vi "test_input_required_result_multi_round.vi"(8 "error in":errorcluster) -> (0 "error out":errorcluster, 3 "text":string)   [LabVIEW 2020, in "Conformance MCP Server.lvlib"]
doc: "Conformance fixture (scenario input-required-result-multi-round). Takes no arguments and asks the user two questions in two rounds with Ask User.vi: first the key step1 (\"Step 1: What is your name?\", a form with the string name), and once that is answered the key step2 (\"Step 2: What is your favorite color?\", a form with the string color). With both answers text is \"Hello, <name>! Your favorite color is <color>.\". While an answer is missing it returns at once and text says which step is open."
uses:
  Conformance MCP Server.lvlib
  <vilib>/JDP Science/JSONtext/Next JSON Value.vi
  <vilib>/JDP Science/JSONtext/String Subset.vi
  <vilib>/JDP Science/JSONtext/support/Strip Quotes and Unescape.vi
  <vilib>/JDP Science/JSONtext/Parsing/Advance past next JSON Value (inlined COPY).vi
  <vilib>/JDP Science/JSONtext/support/Unescape JSON string.vi
  <vilib>/JDP Science/JSONtext/Parsing/Advance past whitespace.vi
  <vilib>/JDP Science/JSONtext/Parsing/Advance past String.vi
  <vilib>/JDP Science/JSONtext/Parsing/Advance past Number.vi
  <vilib>/JDP Science/JSONtext/Parsing/Advance past Line Ending.vi
  <vilib>/JDP Science/JSONtext/Parsing/Parse Full Path or Item Name.vi
  <vilib>/JDP Science/JSONtext/Parsing/Advance past Array.vi
  <vilib>/JDP Science/JSONtext/Parsing/Advance past Object.vi
  <vilib>/JDP Science/JSONtext/support/Error Cluster From Code.vi
  <vilib>/JDP Science/JSONtext/Offset/Find Item Locations by Path.vi
  <vilib>/JDP Science/JSONtext/Parsing/Advance past next JSON Value.vi
  src/MCP Server/MCP Server.lvlib
  <vilib>/JDP Science/JSONtext/JSONtext.lvlib
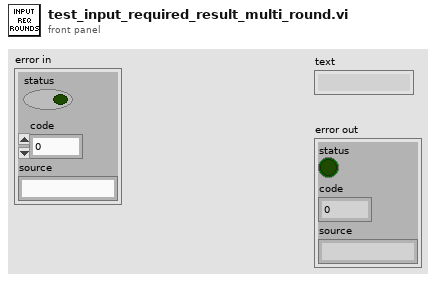
[diagram p1: front panel]
types:
  T1 = enum16{"accept", "decline", "cancel", "pending", "not supported"}
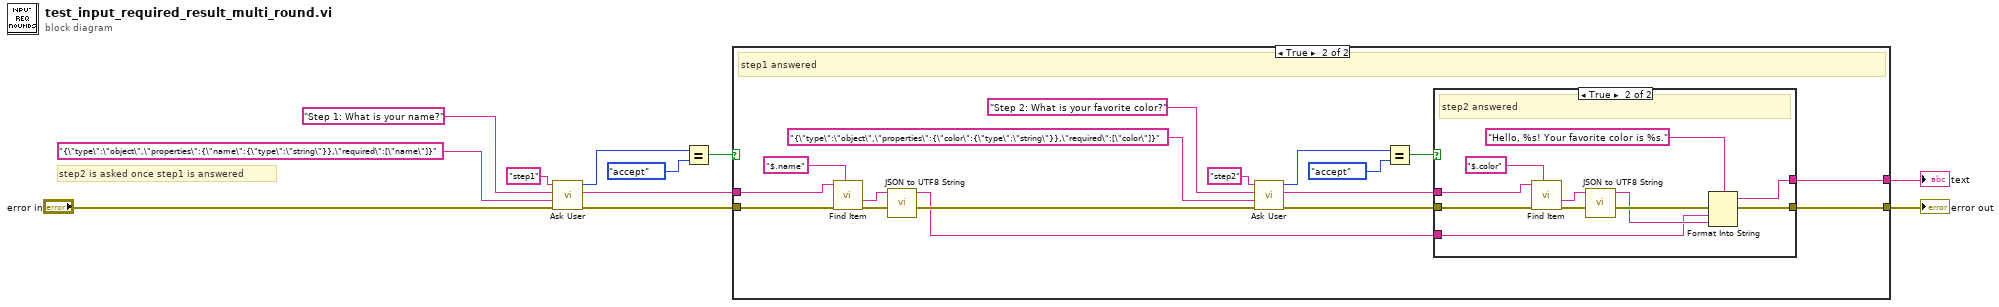
[diagram p0: block diagram]
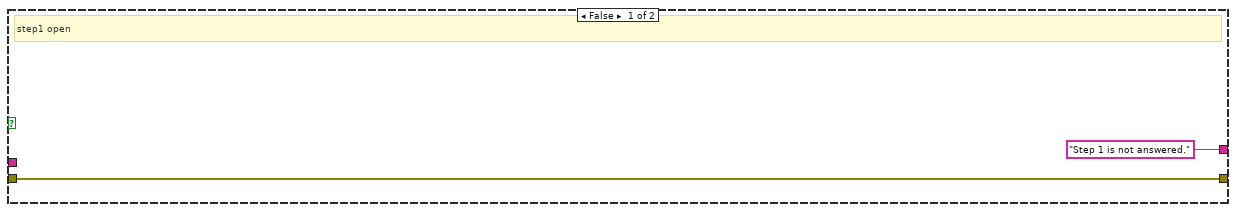
[diagram p2: hidden frame]
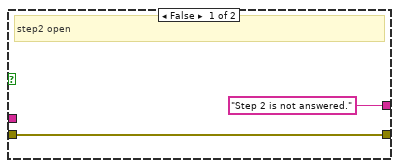
[diagram p3: hidden frame]
diagram:
  # "step2 is asked once step1 is answered"
  n1 = call "Ask User.vi"("error in"="error in", "requestedSchema"="{\"type\":\"object\",\"properties\":{\"name\":{\"type\":\"string\"}},\"required\":[\"name\"]}", "message"="Step 1: What is your name?", "key"="step1") -> ("error out"=w7:errorcluster, "content"=w6:string, "action"=w5:T1)  [unwired: 5 in]
  n2 = Equal?(x=w5, y=T1."accept" ("accept")) -> (x = y?=w9:bool)
  n3 = case shown="True" w9 {
    tunnel: w6 -> [_ w14]
    tunnel: w7 -> [w12 w15]
    tunnel: ["Step 1 is not answered." ("text") w29] -> w10
    tunnel: [w12 w30] -> w11
    frame False {
      # "step1 open"
    }
    frame True {
      # "step1 answered"
      n4 = call <vilib>:"Find Item.vi"("$Path or Item Name"="$.name", "error in (no error)"=w15, "JSON"=w14) -> ("error out"=w17:errorcluster, "<JSON>"=w18:string)  [unwired: 5 in, 2 out]
      n5 = call <vilib>:"JSON to UTF8 String.vi"("error in (no error)"=w17, "JSON"=w18) -> ("error out"=w20:errorcluster, "<UTF8>String"=w19:string)  [unwired: 8 in]
      n6 = call "Ask User.vi"("error in"=w20, "requestedSchema"="{\"type\":\"object\",\"properties\":{\"color\":{\"type\":\"string\"}},\"required\":[\"color\"]}", "message"="Step 2: What is your favorite color?", "key"="step2") -> ("error out"=w26:errorcluster, "content"=w25:string, "action"=w24:T1)  [unwired: 5 in]
      n7 = Equal?(x=w24, y=T1."accept" ("accept")) -> (x = y?=w28:bool)
      n8 = case shown="True" w28 {
        tunnel: w19 -> [_ w35]
        tunnel: w25 -> [_ w33]
        tunnel: w26 -> [w31 w34]
        tunnel: ["Step 2 is not answered." ("text") w42] -> w29
        tunnel: [w31 w43] -> w30
        frame False {
          # "step2 open"
        }
        frame True {
          # "step2 answered"
          n9 = call <vilib>:"Find Item.vi"("$Path or Item Name"="$.color", "error in (no error)"=w34, "JSON"=w33) -> ("error out"=w37:errorcluster, "<JSON>"=w38:string)  [unwired: 5 in, 2 out]
          n10 = call <vilib>:"JSON to UTF8 String.vi"("error in (no error)"=w37, "JSON"=w38) -> ("error out"=w40:errorcluster, "<UTF8>String"=w39:string)  [unwired: 8 in]
          n11 = Format Into String(format string="Hello, %s! Your favorite color is %s.", error in=w40, w35, w39) -> (resulting string=w42:string, error out=w43:errorcluster)  [unwired: 1 in]
        }
      }
    }
  }
  "text" <- w10
  "error out" <- w11
